vi "GetElement(Single).vi"(7 "Qualified Name":string, 8 "error in (no error)":errorcluster, 10 "Key":string, 11 "ConfigManagerCollection in":refnum<class "ConfigManagerCollection.lvclass">) -> (0 "error out":errorcluster, 1 "Value":string, 2 "Key":string, 3 "ConfigManagerCollection out":refnum<class "ConfigManagerCollection.lvclass">, 4 "found":bool)   [LabVIEW 2013, in "CfgManager.lvlib" / "ConfigManagerCollection.lvclass"]
uses:
  ConfigManagerCollection.lvclass
  Manager/ConfigManager.lvclass
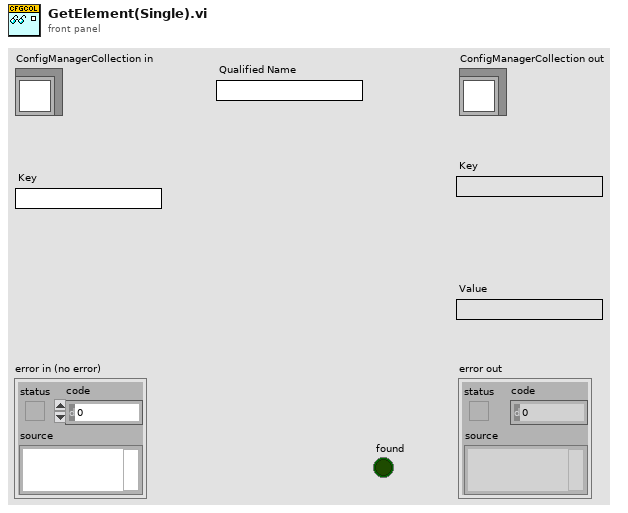
[diagram p1: front panel]
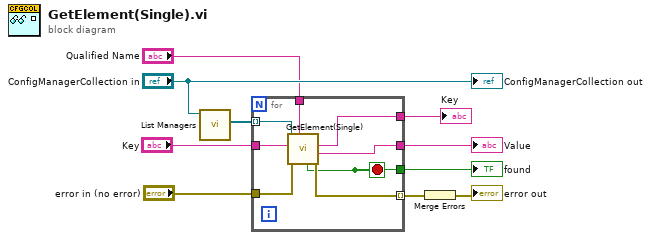
[diagram p0: block diagram]
diagram:
  n1 = call-dynamic "List Managers.vi"("ConfigManagerCollection in"="ConfigManagerCollection in") -> ("List"=w9:refnum<class "ConfigManager.lvclass">[])  [unwired: 9 in, 1 out]
  n2 = for {
    tunnel: w9 -> [w15] mode=indexing
    tunnel: "Key" -> [w18]
    tunnel: "error in (no error)" -> [w17]
    tunnel: [w16] -> w6 mode=indexing
    tunnel: [w13] -> w4
    tunnel: [w12] -> w3
    tunnel: "Qualified Name" -> [w14]
    tunnel: [w11] -> w1
    stop <- w13 stop-if-true
    n3 = call-dynamic "GetElement(Single).vi"("Qualified Name"=w14, "error in (no error)"=w17, "Key"=w18, "ConfigManager in"=w15) -> ("error out"=w16:errorcluster, "Value"=w12:string, "Key"=w11:string, "found"=w13:bool)  [unwired: 3 in, 1 out]
  }
  "Value" <- w3
  "found" <- w4
  "Key" <- w1
  n4 = Merge Errors(w6) -> (→"error out":errorcluster)
  "ConfigManagerCollection out" <- "ConfigManagerCollection in"
